vi "FuncVI-Random.vi"(5 "InstanceRef":T2, 9 "arg list":T1[](array[typedef]) {"num" format="%.2f"}) -> (0 "error out":bool, 3 "result":T1 {"num" format="%.2f"})   [LabVIEW 2021]
doc: "::: CalcExpress Toolkit :::\nCopyright (c) 2000-2026 Konstantin Shifershteyn. All rights reserved."
uses:
  cetypes.llb/CalcExpress Function Argument Info.ctl
  cetypes.llb/CalcExpress Instance RefNum.ctl
panel:
  in  "max arg num":i32=2
  in  "min arg num":i32
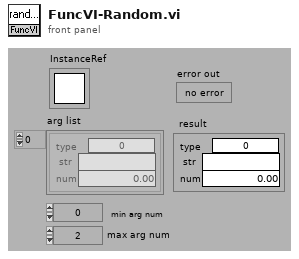
[diagram p1: front panel]
types:
  T1 = typedef "CalcExpress Function Argument Info.ctl" = cluster{"type":u32, "str":string, "num":dbl}
  T2 = typedef "CalcExpress Instance RefNum.ctl" = refnum<k1>
  T3 = enum16{"Array-Array", "Array-Scalar", "Scalar-Array", "Scalar-Scalar"}
  T4 = cluster{"Left 2D":cdb[][], "Left Scalar":cdb, "Right 2D":cdb[][], "Right Scalar":cdb}
  T5 = cluster{"Left 2D":dbl[][], "Left Scalar":dbl, "Right 2D":dbl[][], "Right Scalar":dbl}
  T6 = typedef "CalcExpress Data Type.ctl" = enum32{"String", "DBL Number", "identifier", "1D Array of DBL", "2D Array of DBL", "CDB Number", "1D Array of CDB", "2D Array of CDB", "1D Array of String", "2D Array of String", "Unknown data type"}
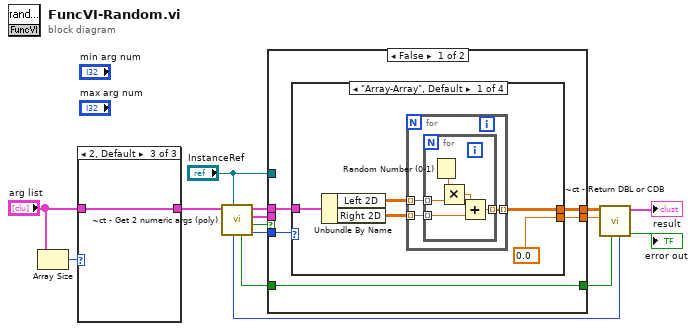
[diagram p0: block diagram]
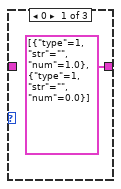
[diagram p2: hidden frame]
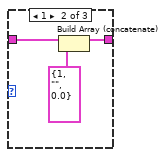
[diagram p3: hidden frame]
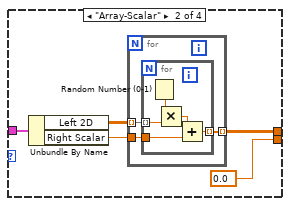
[diagram p4: hidden frame]
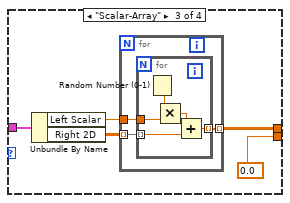
[diagram p5: hidden frame]
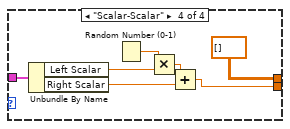
[diagram p6: hidden frame]
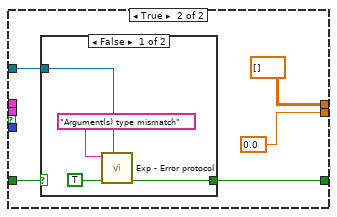
[diagram p7: hidden frame]
diagram:
  n1 = Array Size(array="arg list") -> (size(s)=w3:i32)
  n2 = case shown="2, Default" w3 {
    tunnel: "arg list" -> [_ w19 w20]
    tunnel: [cluster{"type":u8, "str":string, "num":dbl}[] [{"type"=1, "str"="", "num"=1.0}, {"type"=1, "str"="", "num"=0.0}] ("args list") w18 w20] -> w1
    frame 0 {
    }
    frame 1 {
      n3 = Build Array (concatenate)(w19, cluster{"type":u8, "str":string, "num":dbl} {"type"=1, "str"="", "num"=0.0} ("arg info")) -> (w18:T1[])
    }
    frame 2, Default {
    }
  }
  n4 = call "~ct - Get 2 numeric args (poly).vi"("InstanceRef"="InstanceRef", "args list"=w1) -> ("poly"=w9:T3, "CDB ?"=w12:bool, "CDB arguments"=w10:T4, "DBL arguments"=w11:T5, "error out"=w6:bool, "type of result"=w13:T6)  [unwired: 4 in]
  n5 = case shown="False" w12 {
    tunnel: w11 -> [w24 _]
    tunnel: w10 -> [_ _]
    tunnel: w9 -> [w25 _]
    tunnel: [w23 dbl[][] []] -> w8
    tunnel: [w22 0.0] -> w7
    tunnel: w6 -> [w21 w74]
    tunnel: [w21 w73] -> w5
    tunnel: "InstanceRef" -> [_ w72]
    frame False {
      n6 = case shown="\"Array-Array\", Default" w25 {
        tunnel: w24 -> [w30 w43 w56 w71]
        tunnel: [w26 w39 w52 dbl[][] []] -> w23
        tunnel: [0.0 0.0 0.0 w65] -> w22
        frame "Array-Array", Default {
          n7 = Unbundle By Name(w30) -> ("Left 2D"=w28:dbl[][], "Right 2D"=w27:dbl[][])
          n8 = for {
            tunnel: w28 -> [w33] mode=indexing
            tunnel: w27 -> [w32] mode=indexing
            tunnel: [w31] -> w26 mode=indexing
            n9 = for {
              tunnel: w33 -> [w36] mode=indexing
              tunnel: w32 -> [w35] mode=indexing
              tunnel: [w34] -> w31 mode=indexing
              n10 = Random Number (0-1)() -> (number: 0 to 1=w37:dbl)
              n11 = Multiply(x=w37, y=w36) -> (x*y=w38:dbl)
              n12 = Add(x=w38, y=w35) -> (x+y=w34:dbl)
            }
          }
        }
        frame "Array-Scalar" {
          n13 = Unbundle By Name(w43) -> ("Left 2D"=w41:dbl[][], "Right Scalar"=w40:dbl)
          n14 = for {
            tunnel: w41 -> [w46] mode=indexing
            tunnel: w40 -> [w45]
            tunnel: [w44] -> w39 mode=indexing
            n15 = for {
              tunnel: w46 -> [w49] mode=indexing
              tunnel: w45 -> [w48]
              tunnel: [w47] -> w44 mode=indexing
              n16 = Random Number (0-1)() -> (number: 0 to 1=w50:dbl)
              n17 = Multiply(x=w50, y=w49) -> (x*y=w51:dbl)
              n18 = Add(x=w51, y=w48) -> (x+y=w47:dbl)
            }
          }
        }
        frame "Scalar-Array" {
          n19 = Unbundle By Name(w56) -> ("Left Scalar"=w54:dbl, "Right 2D"=w53:dbl[][])
          n20 = for {
            tunnel: w54 -> [w59]
            tunnel: w53 -> [w58] mode=indexing
            tunnel: [w57] -> w52 mode=indexing
            n21 = for {
              tunnel: w59 -> [w62]
              tunnel: w58 -> [w61] mode=indexing
              tunnel: [w60] -> w57 mode=indexing
              n22 = Random Number (0-1)() -> (number: 0 to 1=w63:dbl)
              n23 = Multiply(x=w63, y=w62) -> (x*y=w64:dbl)
              n24 = Add(x=w64, y=w61) -> (x+y=w60:dbl)
            }
          }
        }
        frame "Scalar-Scalar" {
          n25 = Unbundle By Name(w71) -> ("Left Scalar"=w67:dbl, "Right Scalar"=w66:dbl)
          n26 = Random Number (0-1)() -> (number: 0 to 1=w68:dbl)
          n27 = Multiply(x=w68, y=w67) -> (x*y=w69:dbl)
          n28 = Add(x=w69, y=w66) -> (x+y=w65:dbl)
        }
      }
    }
    frame True {
      n29 = case shown="False" w74 {
        selector: w74 -> [_ w81]
        tunnel: [w80 w81] -> w73
        tunnel: w72 -> [w78 _]
        frame False {
          n30 = call "Exp - Error protocol.vi"("InstanceRef"=w78, "error in"=TRUE, "error message in"="Argument(s) type mismatch" ("ErrStr")) -> ("error out"=w80:bool)  [unwired: 5 in, 1 out]
        }
        frame True {
        }
      }
    }
  }
  n31 = call "~ct - Return DBL or CDB.vi"("type"=w13, "error in"=w5, "DBL"=w7, "2D DBL"=w8) -> ("error out"=→"error out":bool, "result"=→"result":T1)  [unwired: 6 in]
